vi "Select_SglVar.vi"(8 "error in (no error)":errorcluster, 10 "varName":string, 11 "muExpr in":refnum<class "mupExpr.lvclass">) -> (0 "error out":errorcluster, 3 "muExpr out":refnum<class "mupExpr.lvclass">)   [LabVIEW 2018, in "mupExpr.lvclass"]
doc: "Select the variable, by name, for use in single variable evaluation.\nReturns error if the input variable is not found."
uses:
  mupExpr.lvclass
  mupExpr.lvclass/mupExpr.ctl
  <vilib>/Utility/error.llb/Error Cluster From Error Code.vi
  <vilib>/ErrorRing/Error Ring.xnode
panel:
  # "Select the variable, by name, for use in single variable evaluation.\nReturns error if the input variable is not found."
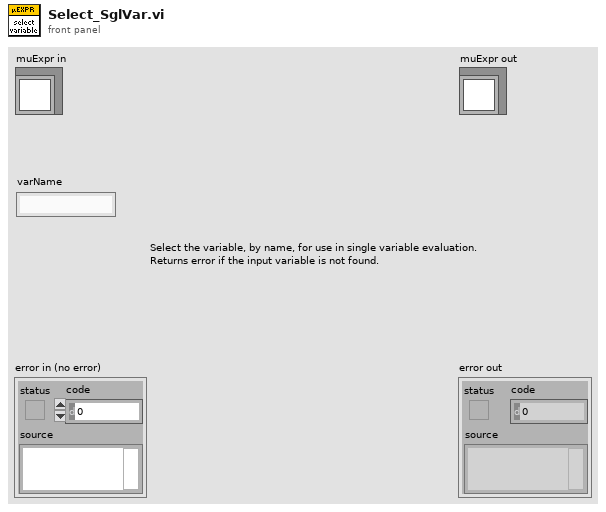
[diagram p1: front panel]
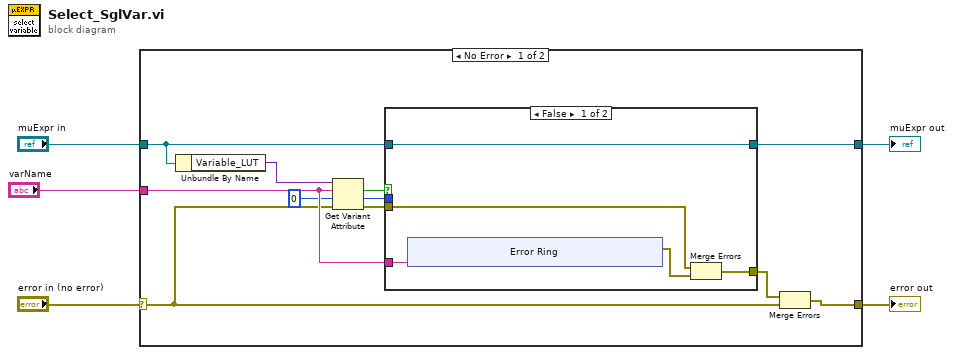
[diagram p0: block diagram]
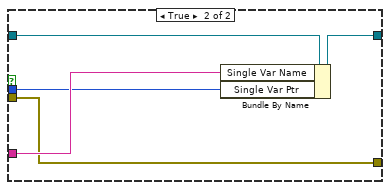
[diagram p2: hidden frame]
diagram:
  n1 = case shown="No Error" "error in (no error)" {
    selector: "error in (no error)" -> [w7 w35]
    tunnel: [w15 w35] -> w4
    tunnel: [w6 w34] -> w2
    tunnel: "muExpr in" -> [w8 w34]
    tunnel: "varName" -> [w16 _]
    frame No Error {
      n2 = Unbundle By Name(w8) -> ("Variable_LUT"=w14:variant)
      n3 = Get Variant Attribute(Variant=w14, name=w16, default value (empty Variant)=u64 0, error in=w7) -> (found=w13:bool, value=w11:u64, error out=w10:errorcluster)  [unwired: 1 out]
      n4 = case shown="False" w13 {
        tunnel: w11 -> [_ w31]
        tunnel: w8 -> [w21 w33]
        tunnel: w16 -> [w18 w32]
        tunnel: [w21 w30] -> w6
        tunnel: w10 -> [w19 w29]
        tunnel: [w20 w29] -> w9
        frame False {
          n5 = xnode "Error Ring"("parameter 0"=w18) -> ("error out"=w17:errorcluster)
          n6 = Merge Errors(w19, w17) -> (w20:errorcluster)
        }
        frame True {
          n7 = Bundle By Name(cluster=w33, "Single Var Name"=w32, "Single Var Ptr"=w31) -> (w30:refnum<class "mupExpr.lvclass">)
        }
      }
      n8 = Merge Errors(w9, w7) -> (w15:errorcluster)
    }
    frame Error {
    }
  }
  "error out" <- w4
  "muExpr out" <- w2
